vi "RemoteVI Track Popups.vi"(0 "look?":bool, 1 "previously hidden":u64[](array[numeric]), 2 "remote click?":bool, 5 "panel hWnd":u64, 7 "d":cluster{"dx":i32, "dy":i32}, 9 "previous popup hWnds":u64[](array[numeric])) -> (3 "hidden hWnds":u64[](array[numeric]), 4 "popups":T2, 6 "overlay popups":T1(array[cluster]), 8 "popup open?":bool, 10 "popup hWnds":u64[](array[numeric]))   [LabVIEW 2020, in "RemoteVI.lvlib"]
doc: "The popup part of one server loop iteration (docs\\architecture.md, Popups). When look? is TRUE the popups are listed (RemoteVI List Popups.vi - Win32 only, no VI Server call); otherwise there are none. Popups a remote user opened are hidden on the host (RemoteVI Hide Remote Popups.vi). popup open? is TRUE when a modal popup (anything but a tip strip or a drop shadow) is open; d is reset to 0, 0 when none is. popups carries the modal popups at their LOGICAL positions (real - d, RemoteVI Logical Popups.vi) for servicing the clients, overlay popups every popup but SysShadow and tip strips for the OVERLAY (the browser shows tip strips itself, from the tips message)."
uses:
  RemoteVI.lvlib
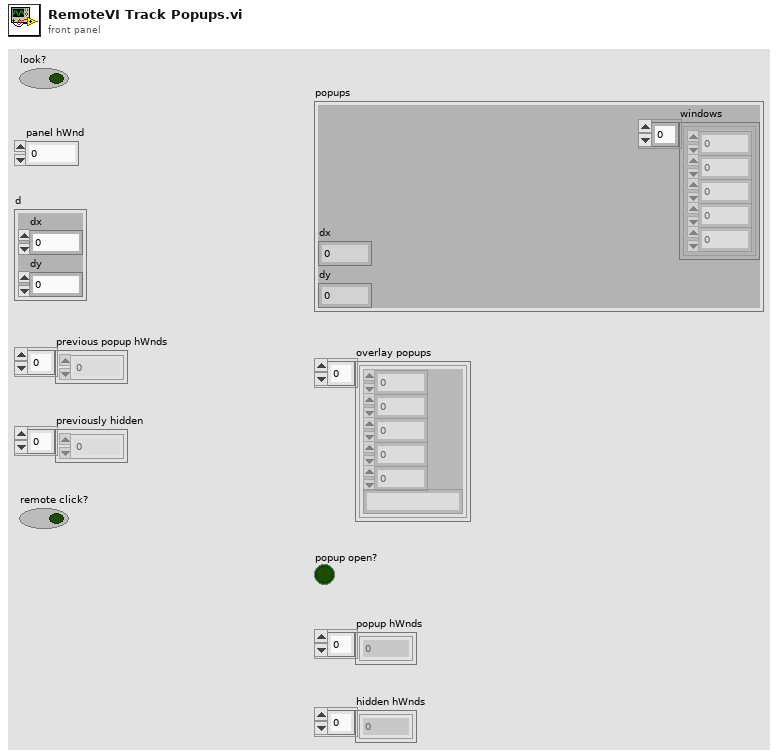
[diagram p1: front panel]
types:
  T1 = cluster{"hwnd":u64, "x":i32, "y":i32, "w":i32, "h":i32, "class":string}[]
  T2 = cluster{"windows":cluster{"hwnd":u64, "x":i32, "y":i32, "w":i32, "h":i32}[], "dx":i32, "dy":i32}
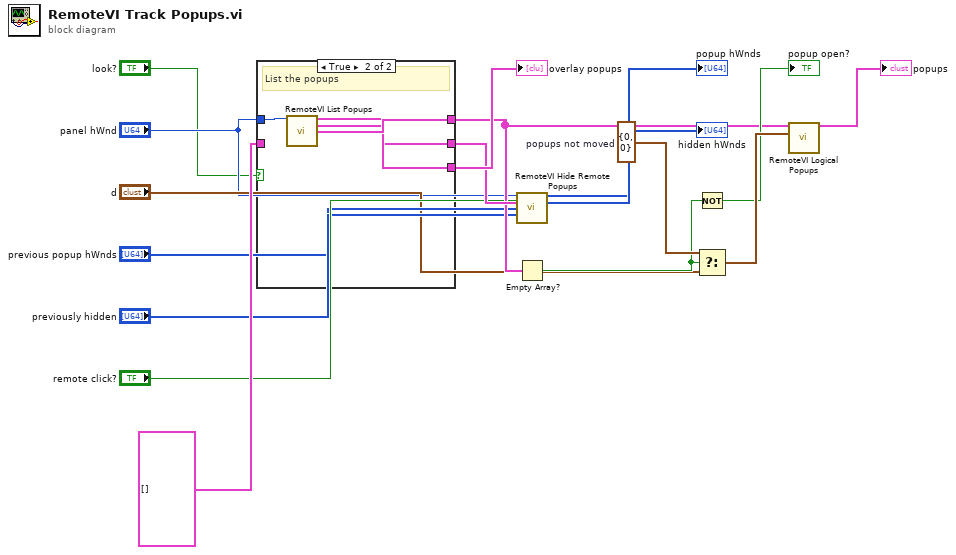
[diagram p0: block diagram]
diagram:
  w15 = cluster{"dx":i32, "dy":i32} {"dx"=0, "dy"=0}  # popups not moved
  n1 = case shown="True" "look?" {
    tunnel: "panel hWnd" -> [_ w19]
    tunnel: T1 [] -> [w18 _]
    tunnel: [w18 w22] -> w8
    tunnel: [w18 w20] -> w9
    tunnel: [w18 w21] -> w10
    frame False {
    }
    frame True {
      # "List the popups"
      n2 = call "RemoteVI List Popups.vi"("panel hWnd"=w19) -> ("all popups"=w20:T1, "overlay popups"=w21:T1, "modal popups"=w22:T1)  [unwired: 12 in]
    }
  }
  "overlay popups" <- w10
  n3 = call "RemoteVI Hide Remote Popups.vi"("panel hWnd"="panel hWnd", "remote click?"="remote click?", "all popups"=w9, "previous popup hWnds"="previous popup hWnds", "previously hidden"="previously hidden") -> ("popup hWnds"=→"popup hWnds":u64[], "hidden hWnds"=→"hidden hWnds":u64[])  [unwired: 9 in]
  n4 = Empty Array?(array=w8) -> (empty?=w13:bool)
  n5 = Not(x=w13) -> (.not. x?=→"popup open?":bool)
  n6 = Select(t=w15, s=w13, f="d") -> (s? t:f=w16:cluster{"dx":i32, "dy":i32})
  n7 = call "RemoteVI Logical Popups.vi"("modal popups"=w8, "d"=w16) -> ("popups"=→"popups":T2)  [unwired: 13 in]
